vi "csb hdlc encode.vi"(7 "frame_cap":i32, 8 "error in (no error)":errorcluster, 9 "frame":u8[](array[numeric]), 10 "len":i32, 11 "payload":u8[](array[numeric])) -> (0 "error out":errorcluster, 1 "frame out":u8[](array[numeric]), 3 "function return":i32)   [LabVIEW 2021, in "CANsub_Codec.lvlib"]
doc: "int32_t csb_hdlc_encode(const uint8_t *payload, int32_t len, uint8_t *frame, int32_t frame_cap);"
uses:
  CANsub_Codec.lvlib
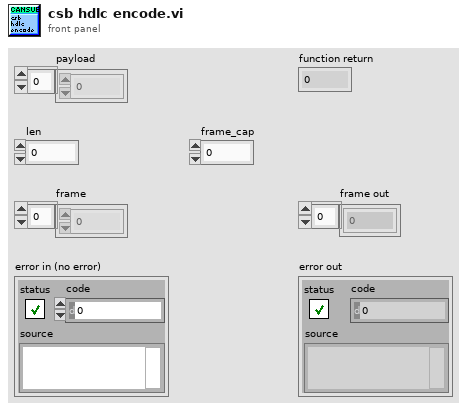
[diagram p1: front panel]
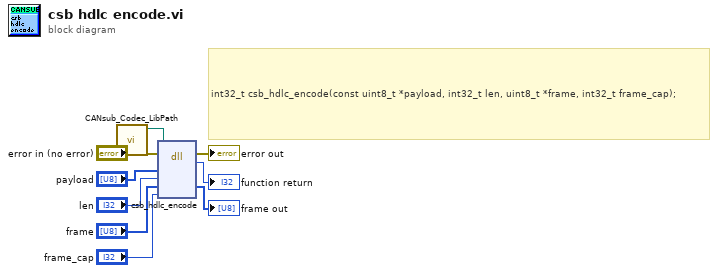
[diagram p0: block diagram]
diagram:
  # "int32_t csb_hdlc_encode(const uint8_t *payload, int32_t len, uint8_t *frame, int32_t frame_cap);"
  n1 = call "CANsub_Codec_LibPath.vi"() -> ("Path"=w1:path)  [unwired: 11 in]
  n2 = dll-call lib="libcansub_codec.*" fn="csb_hdlc_encode"(path in=w1, error in="error in (no error)", "payload"="payload", "len"="len", "frame"="frame", "frame_cap"="frame_cap") -> (error out=→"error out":errorcluster, "return type"=→"function return":i32, "frame"=→"frame out":u8[])  [unwired: 4 in, 1 out]
